vi "FuncVI-viCtrlSet.vi"(5 "InstanceRef":T2, 9 "arg list":T1[](array[typedef]) {"num" format="%.2f"}) -> (0 "error out":bool, 3 "result":T1 {"num" format="%.2f"})   [LabVIEW 2021]
doc: "::: CalcExpress Toolkit :::\nCopyright (c) 2000-2026 Konstantin Shifershteyn. All rights reserved."
uses:
  cetypes.llb/CalcExpress Function Argument Info.ctl
  cetypes.llb/CalcExpress Instance RefNum.ctl
panel:
  in  "max arg num":i32=1000
  in  "min arg num":i32=3
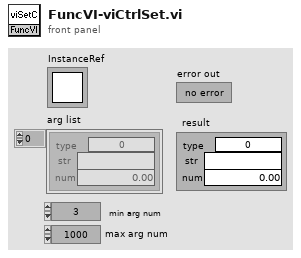
[diagram p1: front panel]
types:
  T1 = typedef "CalcExpress Function Argument Info.ctl" = cluster{"type":u32, "str":string, "num":dbl}
  T2 = typedef "CalcExpress Instance RefNum.ctl" = refnum<k1>
  T3 = enum32{"String", "DBL Number", "identifier", "1D Array of DBL", "2D Array of DBL", "CDB Number", "1D Array of CDB", "2D Array of CDB", "1D Array of String", "2D Array of String", "Unknown data type"}
  T4 = cluster{"index":i32, "data type":enum32{"String", "DBL Number", "identifier", "1D Array of DBL", "2D Array of DBL", "CDB Number", "1D Array of CDB", "2D Array of CDB", "1D Array of String", "2D Array of String", "Unknown data type"}, "default num":dbl, "default str":string}[]
  T5 = cluster{"use this constant to specify a predefined type":enum32{"String", "DBL Number", "identifier", "1D Array of DBL", "2D Array of DBL", "CDB Number", "1D Array of CDB", "2D Array of CDB", "1D Array of String", "2D Array of String", "Unknown data type"}, string, "code":i32}
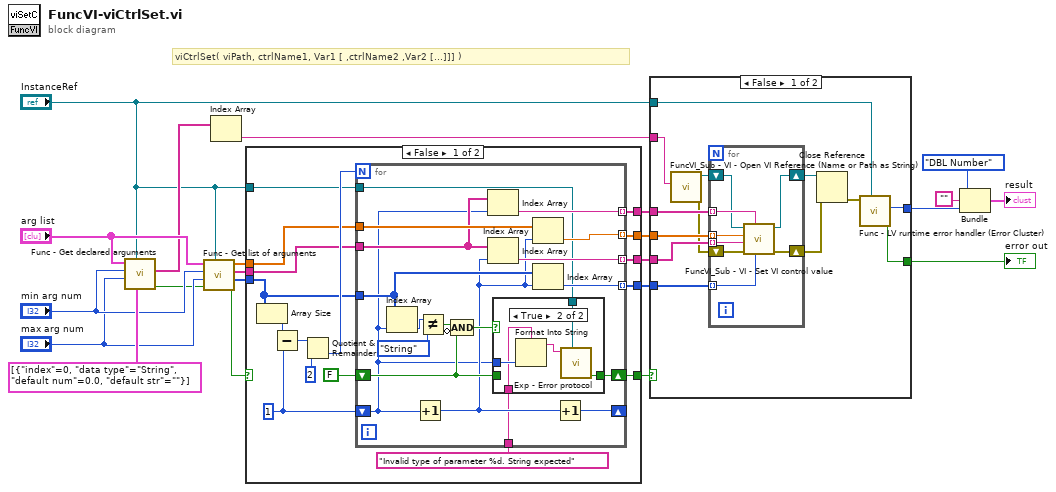
[diagram p0: block diagram]
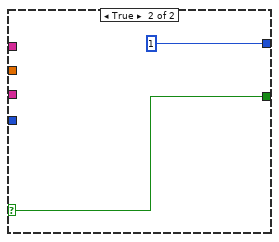
[diagram p2: hidden frame]
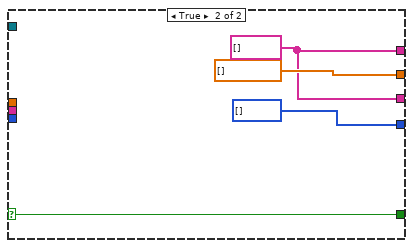
[diagram p4: hidden frame]
diagram:
  # "viCtrlSet( viPath, ctrlName1, Var1 [ ,ctrlName2 ,Var2 [...]]] )"
  n1 = call "Func - Get declared arguments.vi"("arg descriptors"=T4 [{"index"=0, "data type"=enum."String", "default num"=0.0, "default str"=""}] ("args descriptors"), "InstanceRef"="InstanceRef", "max arg num"="max arg num", "min arg num"="min arg num", "arg list"="arg list") -> ("error out"=w14:bool, "str list"=w13:string[])  [unwired: 3 in, 2 out]
  n2 = call "Func - Get list of arguments.vi"("InstanceRef"="InstanceRef", "error in"=w14, "max arg num"="max arg num", "min arg num"="min arg num", "arg list"="arg list") -> ("error out"=w22:bool, "type list"=w19:u32[], "str list"=w20:string[], "num list"=w21:dbl[])  [unwired: 3 in]
  n3 = Index Array(array=w13) -> (element=w1:string)  [unwired: 1 in]
  n4 = case shown="False" w22 {
    selector: w22 -> [_ w66]
    tunnel: [w30 w66] -> w12
    tunnel: w21 -> [w33 _]
    tunnel: w20 -> [w32 _]
    tunnel: w19 -> [w34 _]
    tunnel: [w29 dbl[] []] -> w11
    tunnel: [w28 w63] -> w10
    tunnel: [w27 u32[] []] -> w9
    tunnel: [w26 w63] -> w8
    tunnel: "InstanceRef" -> [w25 _]
    frame False {
      w24 = 1 ("y")
      n5 = Array Size(array=w34) -> (size(s)=w38:i32)
      n6 = Subtract(x=w38, y=w24) -> (x-y=w37:i32)
      n7 = Quotient & Remainder(x=w37, y=2) -> (floor(x/y)=w36:i32)  [unwired: 1 out]
      n8 = for {
        N: w36 -> [_]
        shift-right: [w56] -> _
        shift-left: w24 -> [w40]
        shift-right: [w55] -> w30
        shift-left: FALSE -> [w51]
        tunnel: w34 -> [w48]
        tunnel: w33 -> [w49]
        tunnel: w32 -> [w44]
        tunnel: [w47] -> w27 mode=indexing
        tunnel: [w46] -> w28 mode=indexing
        tunnel: [w45] -> w29 mode=indexing
        tunnel: [w42] -> w26 mode=indexing
        tunnel: "Invalid type of parameter %d. String expected" -> [w41]
        tunnel: w25 -> [w39]
        n9 = Index Array(array=w48, index=w40) -> (element=w54:u32)
        n10 = Increment(x=w40) -> (x+1=w43:i32)
        n11 = Not Equal?(x=w54, y=T3."String") -> (x != y?=w52:bool)
        n12 = Compound Arithmetic op=AND(w52, invert w51) -> (w50:bool)
        n13 = Index Array(array=w44, index=w40) -> (element=w42:string)
        n14 = Index Array(array=w44, index=w43) -> (element=w46:string)
        n15 = case shown="True" w50 {
          tunnel: [w57 w62] -> w55
          tunnel: w51 -> [w57 _]
          tunnel: w40 -> [_ w60]
          tunnel: w41 -> [_ w59]
          tunnel: w39 -> [_ w58]
          frame False {
          }
          frame True {
            n16 = Format Into String(format string=w59, w60) -> (resulting string=w61:string)  [unwired: 2 in, 1 out]
            n17 = call "Exp - Error protocol.vi"("InstanceRef"=w58, "error message in"=w61) -> ("error out"=w62:bool)  [unwired: 6 in, 1 out]
          }
        }
        n18 = Index Array(array=w49, index=w43) -> (element=w45:dbl)
        n19 = Index Array(array=w48, index=w43) -> (element=w47:u32)
        n20 = Increment(x=w43) -> (x+1=w56:i32)
      }
    }
    frame True {
      w63 = string[] []
    }
  }
  n21 = case shown="False" w12 {
    selector: w12 -> [_ w89]
    tunnel: w11 -> [w79 _]
    tunnel: w10 -> [w78 _]
    tunnel: w9 -> [w77 _]
    tunnel: w8 -> [w76 _]
    tunnel: w1 -> [w72 _]
    tunnel: [w67 w89] -> w6
    tunnel: "InstanceRef" -> [w69 _]
    tunnel: [w68 1 ("code")] -> w3
    frame False {
      n22 = call "FuncVI_Sub - VI - Open VI Reference (Name or Path as String).vi"("VI name or path"=w72) -> ("error out"=w74:errorcluster, "VI Refnum"=w75:refnum<vi>)  [unwired: 9 in]
      n23 = for {
        tunnel: w79 -> [w87] mode=indexing
        tunnel: w78 -> [w86] mode=indexing
        tunnel: w77 -> [w85] mode=indexing
        tunnel: w76 -> [w84] mode=indexing
        shift-right: [w82] -> w70
        shift-left: w74 -> [w83]
        shift-right: [w81] -> w71
        shift-left: w75 -> [w80]
        n24 = call "FuncVI_Sub - VI - Set VI control value.vi"("type"=w85, "control name"=w84, "error in"=w83, "str"=w86, "dbl"=w87, "VI Ref"=w80) -> ("error out"=w82:errorcluster, "dup VI Ref"=w81:refnum<vi>)  [unwired: 4 in]
      }
      n25 = Close Reference(reference=w71, error in (no error)=w70) -> (error out=w73:errorcluster)
      n26 = call "Func - LV runtime error handler (Error Cluster).vi"("InstanceRef"=w69, "LabVIEW error"=w73) -> ("error out"=w67:bool, "LV error code"=w68:i32)  [unwired: 4 in, 2 out]
    }
    frame True {
    }
  }
  "error out" <- w6
  n27 = Bundle("use this constant to specify a predefined type"=T3."DBL Number", "", "code"=w3) -> (→"result":T5)  [unwired: 1 in]
